vi "Untitled 1.vi"() -> ()   [LabVIEW 2025]
uses:
  <vilib>/addons/control/pid/NI_PID_autopid.lvlib
  <vilib>/gmath/NI_Gmath.lvlib
panel:
  in  "x":dbl format="%0.2f"
  out "Waveform Chart 2":dynamicdata(graph)
  in  "stop":bool
  out "Waveform Chart":dbl(graph)
  out "tuning completed?":bool
  out "output":dbl format="%.2f"
  in  "autotune? (F) 2":bool
  in  "PID gains 2":T1={"proportional gain (Kc)"=1.0, "integral time (Ti, min)"=0.01, "derivative time (Td, min)"=0.0} {"derivative time (Td, min)" format="%.3f"; "integral time (Ti, min)" format="%.3f"; "proportional gain (Kc)" format="%.3f"}
  out "process variable 2":dbl format="%.2f"
  out "setpoint 2":dbl format="%#_13g"
  in  "output range 2":cluster{"output high":dbl, "output low":dbl}={"output high"=100.0, "output low"=-100.0} {"output low" format="%.2f"; "output high" format="%.2f"}
  in  "autotuning parameters 2":T2={"controller type"=1, "relay cycles"=3, "relay amplitude"=1.0, "control specification"=2, "PV noise level"=0.1} {"PV noise level" format="%.2f"; "control specification" items=["normal", "fast", "slow"]; "relay amplitude" format="%.2f"; "controller type" items=["PID", "PI", "P"]}
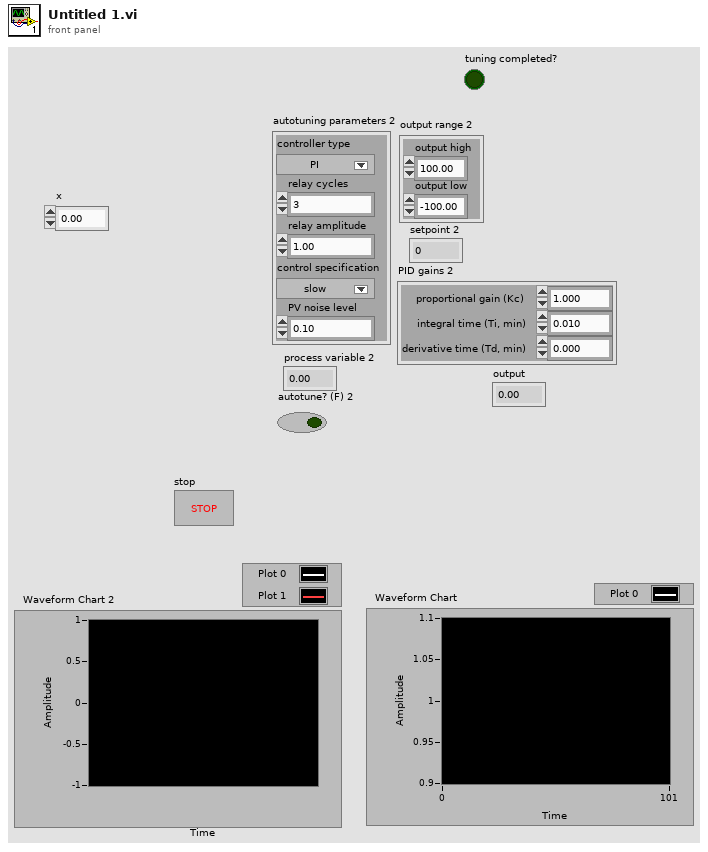
[diagram p1: front panel]
types:
  T1 = cluster{"proportional gain (Kc)":dbl, "integral time (Ti, min)":dbl, "derivative time (Td, min)":dbl}
  T2 = cluster{"controller type":u16, "relay cycles":i32, "relay amplitude":dbl, "control specification":u16, "PV noise level":dbl}
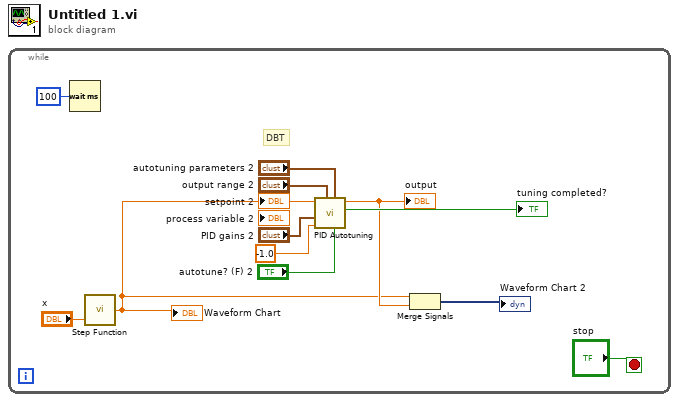
[diagram p0: block diagram]
diagram:
  n1 = while {
    stop <- "stop" stop-if-true
    # "DBT"
    n2 = Wait (ms)(milliseconds to wait=u32 100) -> ()  [unwired: 1 out]
    n3 = call <vilib>:"Step Function.vi"("x"="x") -> ("step(x)"=w1:dbl)
    "setpoint 2" <- w1
    "Waveform Chart" <- w1
    n4 = call <vilib>:"PID Autotuning.vi"("autotune? (F)"="autotune? (F) 2", "autotuning parameters"="autotuning parameters 2", "output range"="output range 2", "dt (s)"=-1.0, "PID gains"="PID gains 2", "setpoint"=w1) -> ("tuning completed?"=→"tuning completed?":bool, "output"=w4:dbl)  [unwired: 2 in, 2 out]
    "output" <- w4
    n5 = Merge Signals(w1, w4) -> (→"Waveform Chart 2":dynamicdata)
  }
